vi "VIH HelpGen - Write HTML File - Common - Author Info.vi"(4 "Product Info Template":string, 6 "Product Info":T3, 7 "Save params":T1, 8 "error in":errorcluster, 10 "HTML in":string, 11 "VI Reference":refnum<vi>) -> (0 "error out":errorcluster, 2 "HTML out":string, 3 "dup VI Reference":refnum<vi>)   [LabVIEW 2014]
doc: "::: VI Helpeks :::\nCopyright (c) 2000-2026 Konstantin Shifershteyn. All rights reserved."
uses:
  VIH HelpGen Typedef - Enum - Default,Enable,Disable.ctl
panel:
  # "VI Helpeks\nCopyright (c) 2012-2026 Konstantin Shifershteyn"
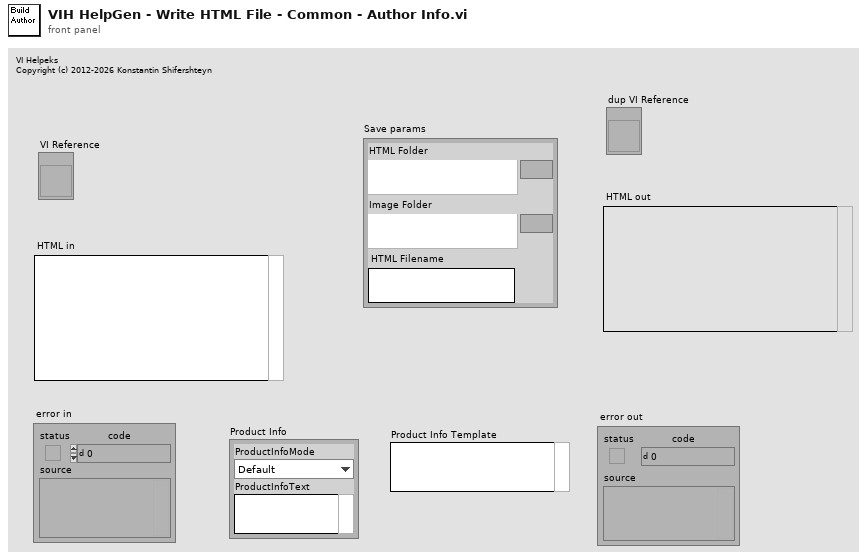
[diagram p1: front panel]
types:
  T1 = cluster{"HTML Folder":path, "Image Folder":path, "HTML Filename":string}
  T2 = typedef "VIH HelpGen Typedef - Enum - Default,Enable,Disable.ctl" = enum16{"Default", "Enable", "Disable"}
  T3 = cluster{"ProductInfoMode":T2, "ProductInfoText":string}
  T4 = enum16{"none", "LV description", "VH minimum", "VH extended"}
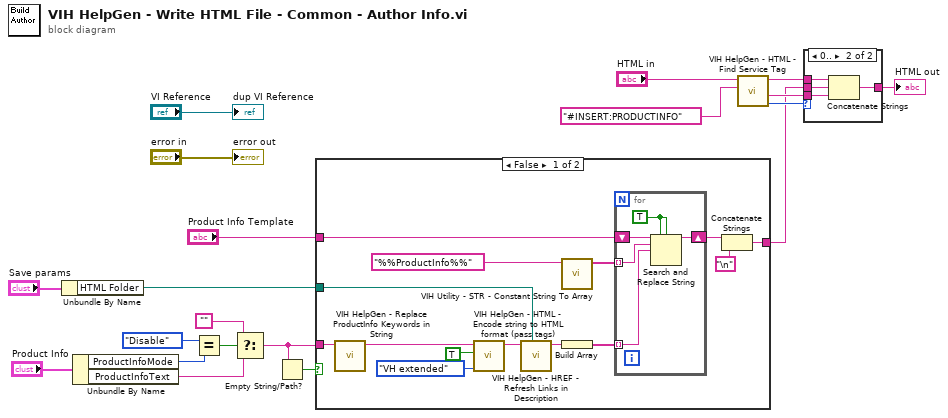
[diagram p0: block diagram]
diagram:
  n1 = Unbundle By Name("Save params") -> ("HTML Folder"=w1:path)
  n2 = Unbundle By Name("Product Info") -> ("ProductInfoMode"=w8:T2, "ProductInfoText"=w5:string)
  n3 = Equal?(x=VIH_HelpGen_Typedef_-_Enum_-_Default,Enable,Disable."Disable", y=w8) -> (x = y?=w6:bool)
  n4 = Select(t="", s=w6, f=w5) -> (s? t:f=w3:string)
  n5 = Empty String/Path?(string/path=w3) -> (empty?=w12:bool)
  n6 = case shown="False" w12 {
    tunnel: [w21 _] -> w13
    tunnel: w3 -> [w25 _]
    tunnel: "Product Info Template" -> [w31 _]
    tunnel: w1 -> [w26 _]
    frame False {
      n7 = call "VIH HelpGen - Replace ProductInfo Keywords in String.vi"("String in"=w25) -> ("String out"=w24:string)  [unwired: 10 in]
      n8 = call "VIH HelpGen - HTML - Encode string to HTML format (pass tags).vi"("HTML Tagset allowed"=T4."VH extended", "Reject CR (F)"=TRUE, "string"=w24) -> ("HTML string"=w28:string)  [unwired: 8 in]
      n9 = call "VIH HelpGen - HREF - Refresh Links in Description.vi"("HTML Folder"=w26, "Description in"=w28) -> ("Description out"=w27:string)  [unwired: 9 in]
      n10 = call "VIH Utility - STR - Constant String To Array.vi"("String in"="%%ProductInfo%%") -> ("Array out"=w33:string[])  [unwired: 10 in]
      n11 = Build Array(w27) -> (w32:string[])
      n12 = for {
        shift-right: [w38] -> w22
        shift-left: w31 -> [w39]
        tunnel: w33 -> [w36] mode=indexing
        tunnel: w32 -> [w35] mode=indexing
        w37 = TRUE
        n13 = Search and Replace String(replace all?=w37, case sensitive?=w37, input string=w39, search string=w36, replace string=w35) -> (result string=w38:string)  [unwired: 3 in, 3 out]
      }
      n14 = Concatenate Strings(w22, "\n") -> (w21:string)
    }
    frame True {
    }
  }
  n15 = call "VIH HelpGen - HTML - Find Service Tag.vi"("Tag name"="#INSERT:PRODUCTINFO", "HTML in"="HTML in") -> ("Offset out"=w16:i32, "After"=w17:string, "Before"=w18:string)  [unwired: 6 in, 1 out]
  n16 = case shown="0.." w16 {
    tunnel: w18 -> [w40 w44]
    tunnel: w17 -> [_ w43]
    tunnel: [w40 w42] -> w10
    tunnel: w13 -> [_ w41]
    frame ..-1 {
    }
    frame 0.. {
      n17 = Concatenate Strings(w44, w41, w43) -> (w42:string)
    }
  }
  "HTML out" <- w10
  "error out" <- "error in"
  "dup VI Reference" <- "VI Reference"
